vi "A_del.vi"(11 "Filename":string) -> (1 "before substring 2":string, 2 "after substring 4":string, 3 "after substring":string)   [LabVIEW 2018]
panel:
  out "before substring":string
  out "after substring 3":string
  out "after substring 2":string
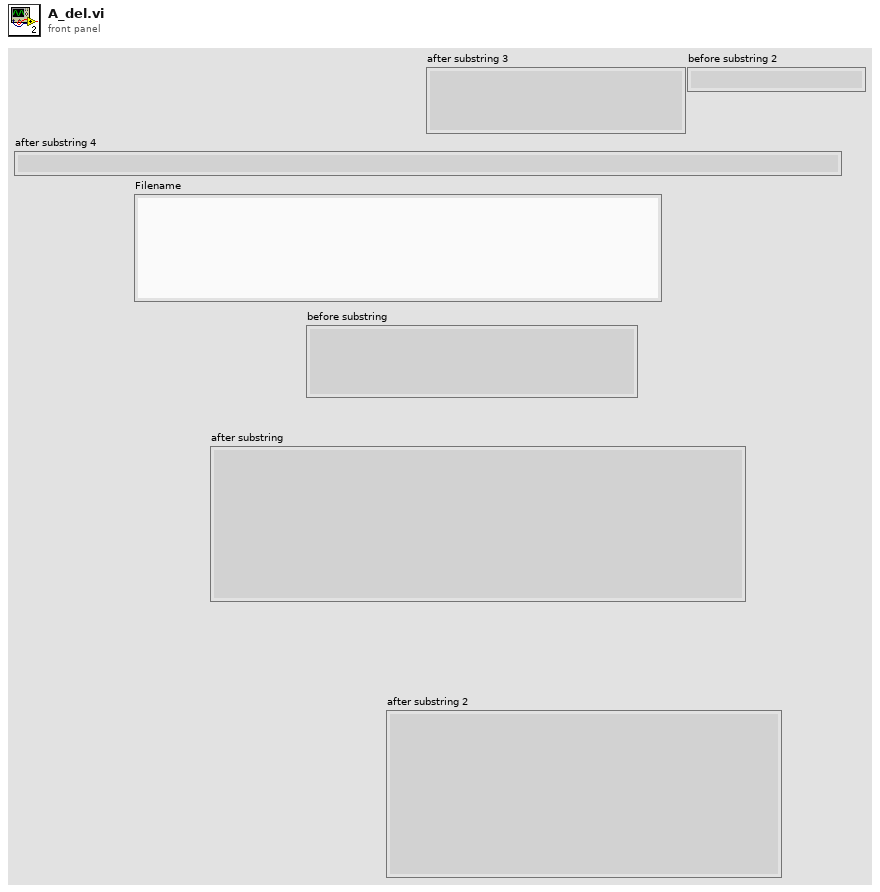
[diagram p1: front panel]
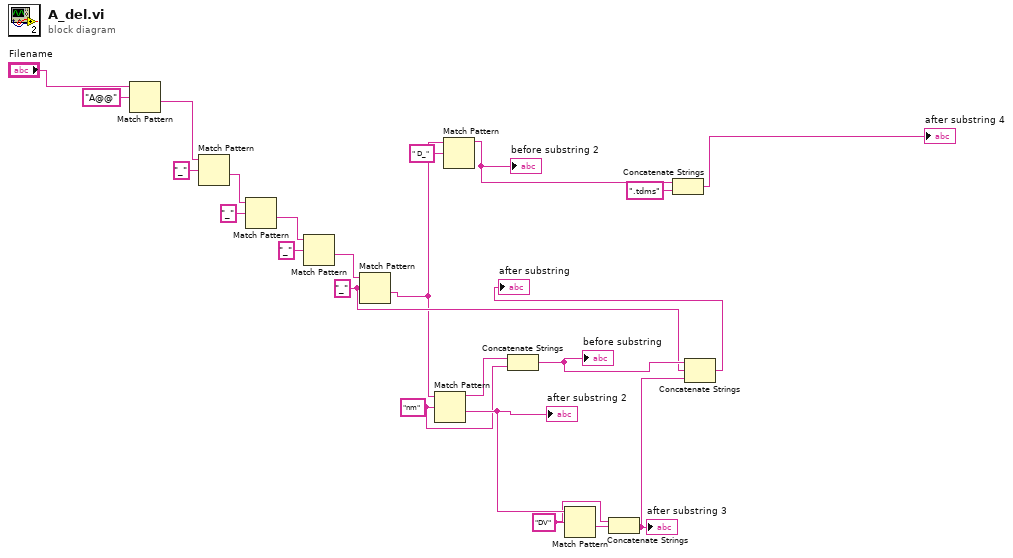
[diagram p0: block diagram]
diagram:
  w11 = "DV" ("regular expression")
  w12 = "nm" ("regular expression")
  w9 = "_" ("regular expression")
  n1 = Match Pattern(string="Filename", regular expression="A@@") -> (after substring=w19:string)  [unwired: 1 in, 3 out]
  n2 = Match Pattern(string=w19, regular expression="_") -> (after substring=w6:string)  [unwired: 1 in, 3 out]
  n3 = Match Pattern(string=w6, regular expression="_") -> (after substring=w17:string)  [unwired: 1 in, 3 out]
  n4 = Match Pattern(string=w17, regular expression="_") -> (after substring=w16:string)  [unwired: 1 in, 3 out]
  n5 = Match Pattern(string=w16, regular expression=w9) -> (after substring=w5:string)  [unwired: 1 in, 3 out]
  n6 = Match Pattern(string=w5, regular expression=w12) -> (before substring=w13:string, after substring=w15:string)  [unwired: 1 in, 2 out]
  "after substring 2" <- w15
  n7 = Match Pattern(string=w5, regular expression=" D_") -> (before substring=w3:string)  [unwired: 1 in, 3 out]
  "before substring 2" <- w3
  n8 = Concatenate Strings(w13, w12) -> (w10:string)
  "before substring" <- w10
  n9 = Match Pattern(string=w15, regular expression=w11) -> (after substring=w14:string)  [unwired: 1 in, 3 out]
  n10 = Concatenate Strings(w11, w14) -> (w8:string)
  "after substring 3" <- w8
  n11 = Concatenate Strings(w3, ".tdms" ("string")) -> (→"after substring 4":string)
  n12 = Concatenate Strings(w10, w9, w8) -> (→"after substring":string)
